vi "NR check Center Channel.vi"(8 "error in (no error)":errorcluster caption="에러 입력(에러 없음)", 10 "Center Channel Number":u32, 11 "Instrument Manager 입력":refnum<class "Instrument Manager.lvclass">) -> (0 "error out":errorcluster caption="에러 출력", 2 "Success?":bool, 3 "Instrument Manager 출력":refnum<class "Instrument Manager.lvclass">)   [LabVIEW 2023, in "Instrument Manager.lvclass"]
uses:
  Instrument Manager.lvclass
  Module/ANRITSU Call Box/Type Definition/Uplink Downlink Enum.ctl
  Module/ANRITSU Call Box/Type Definition/NR Selected CC Type Arguments.ctl
  Instrument Manager.lvclass/Instrument Manager.ctl
  Module/ANRITSU Call Box/Interface Class/Anritsu Call Box.lvclass
  Module/ANRITSU Call Box/ANRITSU Call Box.lvlib
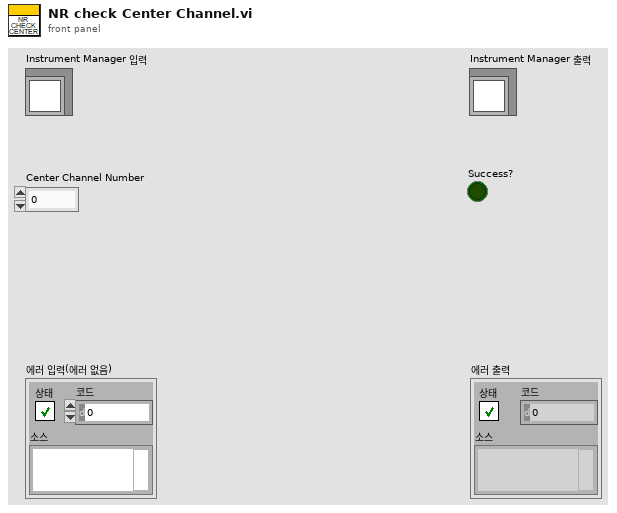
[diagram p1: front panel]
types:
  T1 = typedef "ANRITSU Call Box.lvlib/Uplink Downlink Enum.ctl" = enum16{"Uplink", "Downlink"}
  T2 = typedef "ANRITSU Call Box.lvlib/NR Selected CC Type Arguments.ctl" = cluster{"Selected CC":enum16{"PCC", "SCC", "FR2_PCC", "FR2_SCC"}, "SCC or FR2_SCC Index":u32}
  T3 = cluster{"Anritsu Call Box":refnum<class "Anritsu Call Box.lvclass">, "Spectrum Analyzer":refnum<class "Interface_Spectrum.lvclass">, "RF Switch Box":refnum<class "RF Filter Box.lvclass">, "Turn Table":refnum<class "Interface - Turn Table.lvclass">, "Mast":refnum<class "Interface - Mast.lvclass">, "3D Controller":refnum<class "Interface_3D Controller.lvclass">}
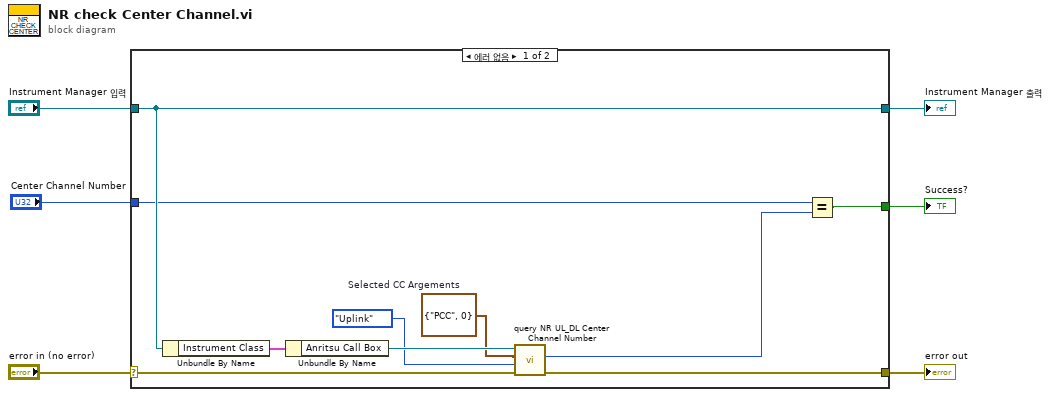
[diagram p0: block diagram]
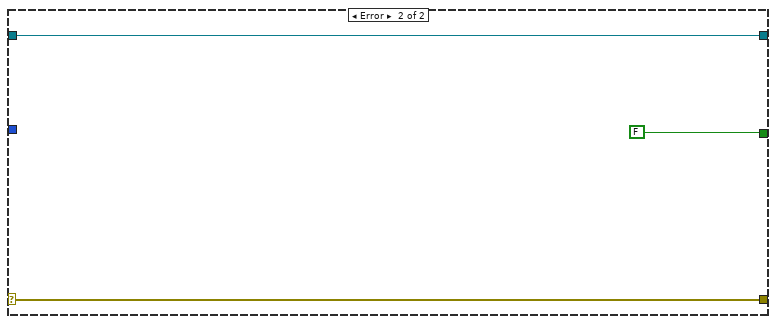
[diagram p2: hidden frame]
diagram:
  n1 = case shown="에러 없음" "error in (no error)" {
    selector: "error in (no error)" -> [w16 w19]
    tunnel: [w15 w19] -> w5
    tunnel: [w14 w18] -> w3
    tunnel: "Instrument Manager 입력" -> [w14 w18]
    tunnel: "Center Channel Number" -> [w8 _]
    tunnel: [w7 FALSE] -> w1
    frame No Error {
      w10 = T2 {"Selected CC"=enum."PCC", "SCC or FR2_SCC Index"=0}  # Selected CC Argements
      n2 = Unbundle By Name(w14) -> ("Instrument Class"=w13:T3)
      n3 = Unbundle By Name(w13) -> ("Anritsu Call Box"=w12:refnum<class "Anritsu Call Box.lvclass">)
      n4 = call-dynamic "query NR UL_DL Center Channel Number.vi"("error in (no error)"=w16, "Direction"=Uplink_Downlink_Enum."Uplink", "Selected CC Argements"=w10, "Anritsu Call Box in"=w12) -> ("error out"=w15:errorcluster, "Center Channel Number"=w9:u32)  [unwired: 5 in, 1 out]
      n5 = Equal?(x=w8, y=w9) -> (x = y?=w7:bool)
    }
    frame Error {
    }
  }
  "error out" <- w5
  "Instrument Manager 출력" <- w3
  "Success?" <- w1
